vi "[ex ce] Signal Generation.vi"() -> ()   [LabVIEW 2021]
doc: "This simple example VI demonstrates a use of CalcExpress for signal generation. Resulting signal is played on a sound output device.\n\nYou need the <B>LabVIEW Advanced Analysis VIs</B> to run some scripts in this example VI.\n\n::: CalcExpress Toolkit :::\nCopyright (c) 2000-2026 Konstantin Shifershteyn. All rights reserved."
uses:
  <vilib>/sound2/lvsound2.llb/Sound Data Format.ctl
  <vilib>/sound2/lvsound2.llb/Sound Output Write (DBL Single).vi
panel:
  out "graph":dbl[](graph)
  in  "result variable":string="out"
  in  "Sound Rate (Hz) : rate":enum16{"11025", "22050", "44100"}(ring)
  in  "Sound device":u32
  in  "script selector":u16(ring) items=["***  Click here to select an example script  ***", "Sine Wave", "Beeper", "Damped oscillations"]
  in  "script":string="/*\nStart this VI and select an example script in the ring above for placing it into this text box.\n\nClick Exec button to process a script.\n*/\n"
  in  "stop":bool
  # "NOTE. Some functions of this example use Advanced Analysis VIs.\nThe example doesn't work properly if you don't have these VIs."
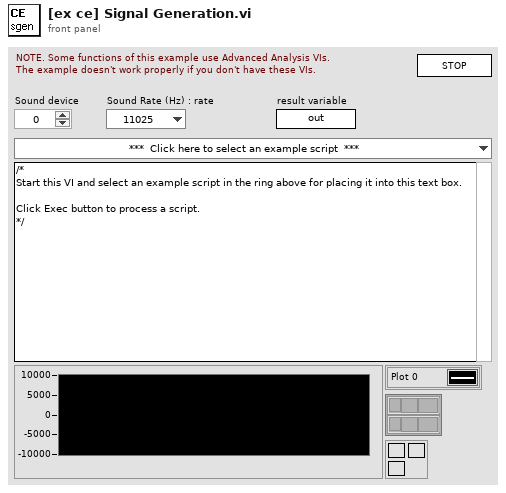
[diagram p1: front panel]
types:
  T1 = typedef "Sound Data Format.ctl" = cluster{"sample rate (S/s)":dbl, "number of channels":i32, "bits per sample":i32}
  T2 = enum16{"create", "destroy", "set value", "get value"}
  T3 = typedef "VarMan Variable Context Handle.ctl" = i32
  T4 = typedef "Sound Output Task ID.ctl" = u32
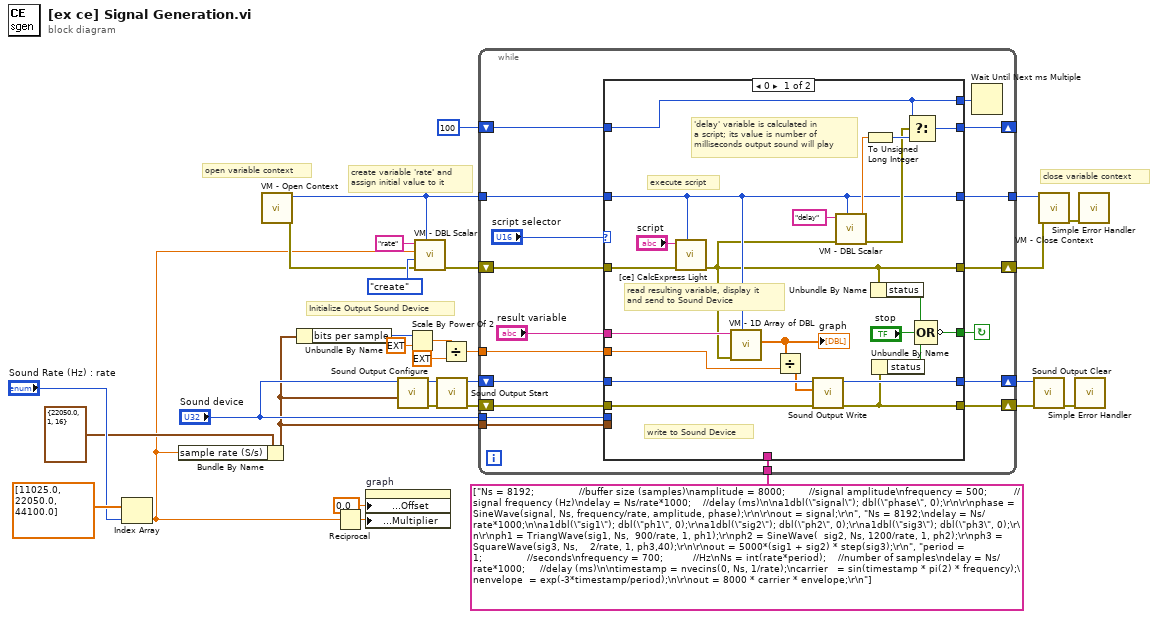
[diagram p0: block diagram]
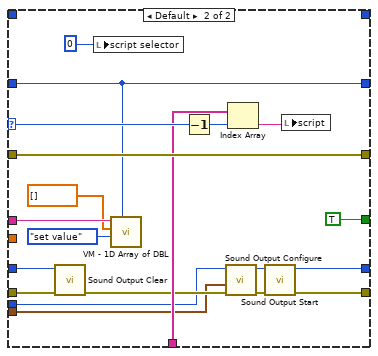
[diagram p2: hidden frame]
diagram:
  # "Initialize Output Sound Device"
  # "close variable context"
  # "create variable 'rate' and\nassign initial value to it"
  # "open variable context"
  n1 = Index Array(array=dbl[] [11025.0, 22050.0, 44100.0], index="Sound Rate (Hz) : rate") -> (element=w8:dbl)
  n2 = Bundle By Name(cluster=T1 {"sample rate (S/s)"=22050.0, "number of channels"=1, "bits per sample"=16} ("sound format"), "sample rate (S/s)"=w8) -> (w1:T1)
  n3 = call "VM - Open Context.vi"() -> ("error out"=w10:errorcluster, "VC Handle out"=w11:T3)  [unwired: 9 in, 1 out]
  n4 = Unbundle By Name(w1) -> ("bits per sample"=w7:i32)
  n5 = Reciprocal(x=w8) -> (1/x=w16:dbl)
  n6 = property on="graph" class="WFGraph (strict)"("X Scale.Offset and Multiplier:Offset"=0.0 ("Xo"), "X Scale.Offset and Multiplier:Multiplier"=w16) -> ()  [unwired: 2 in, 2 out]
  n7 = call <vilib>:"Sound Output Configure.vi"("sound format"=w1, "device ID"="Sound device") -> ("error out"=w19:errorcluster, "task ID"=w22:T4)  [unwired: 8 in]
  n8 = Scale By Power Of 2(n=w7, x=ext 1.0) -> (x*2^n=w5:ext)
  n9 = call "VM - DBL Scalar.vi"("VC Handle"=w11, "error in"=w10, "cmd"=T2."create", "value in"=w8, "name_spec"="rate" ("name")) -> ("error out"=w29:errorcluster)  [unwired: 1 in, 5 out]
  n10 = call <vilib>:"Sound Output Start.vi"("error in (no error)"=w19, "task ID"=w22) -> ("error out"=w20:errorcluster, "task ID out"=w21:T4)  [unwired: 8 in]
  n11 = Divide(x=w5, y=ext 2.0) -> (x/y=w4:ext)
  n12 = while {
    tunnel: string[] ["Ns = 8192;               //buffer size (samples)\namplitude = 8000;        //signal amplitude\nfrequency = 500;         //signal frequency (Hz)\ndelay = Ns/rate*1000;    //delay (ms)\n\na1dbl(\"signal\"); dbl(\"phase\", 0);\r\n\r\nphase = SineWave(signal, Ns, frequency/rate, amplitude, phase);\r\n\r\nout = signal;\r\n", "Ns = 8192;\ndelay = Ns/rate*1000;\n\na1dbl(\"sig1\"); dbl(\"ph1\", 0);\r\na1dbl(\"sig2\"); dbl(\"ph2\", 0);\r\na1dbl(\"sig3\"); dbl(\"ph3\", 0);\r\n\r\nph1 = TriangWave(sig1, Ns,  900/rate, 1, ph1);\r\nph2 = SineWave(  sig2, Ns, 1200/rate, 1, ph2);\r\nph3 = SquareWave(sig3, Ns,    2/rate, 1, ph3,40);\r\n\r\nout = 5000*(sig1 + sig2) * step(sig3);\r\n", "period = 1;               //seconds\nfrequency = 700;          //Hz\nNs = int(rate*period);    //number of samples\ndelay = Ns/rate*1000;     //delay (ms)\n\ntimestamp = nvecins(0, Ns, 1/rate);\ncarrier   = sin(timestamp * pi(2) * frequency);\nenvelope  = exp(-3*timestamp/period);\n\r\nout = 8000 * carrier * envelope;\r\n"] -> [w38]
    shift-left: u32 100 -> [w40]
    shift-right: [w41] -> _
    shift-left: w20 -> [w35]
    shift-right: [w43] -> w23
    tunnel: w11 -> [w47]
    tunnel: [w44] -> w30
    shift-left: w29 -> [w46]
    shift-right: [w42] -> w14
    tunnel: w4 -> [w37]
    shift-right: [w45] -> w24
    shift-left: w21 -> [w36]
    tunnel: "Sound device" -> [w33]
    tunnel: w1 -> [w32]
    stop <- w48 continue-if-true
    n13 = case shown="0" "script selector" {
      selector: "script selector" -> [_ w87]
      tunnel: [w70 TRUE] -> w48
      tunnel: w47 -> [w50 w74]
      tunnel: w46 -> [w68 w90]
      tunnel: w36 -> [w67 w82]
      tunnel: w35 -> [w66 w81]
      tunnel: [w65 w78] -> w45
      tunnel: [w50 w74] -> w44
      tunnel: [w63 w79] -> w43
      tunnel: [w49 w90] -> w42
      tunnel: [w58 _] -> w41
      tunnel: w40 -> [w57 _]
      tunnel: [w57 _] -> w39
      tunnel: w38 -> [_ w85]
      tunnel: w37 -> [w53 _]
      tunnel: w33 -> [_ w77]
      tunnel: w32 -> [_ w76]
      tunnel: "result variable" -> [w51 w75]
      frame 0 {
        # "'delay' variable is calculated in\na script; its value is number of\nmilliseconds output sound will play"
        # "read resulting variable, display it\nand send to Sound Device"
        # "execute script"
        # "write to Sound Device"
        n14 = call "[ce] CalcExpress Light.vi"("VC Handle"=w50, "error in"=w68, "expression"="script") -> ("error out"=w49:errorcluster)  [unwired: 6 in, 2 out]
        n15 = call "VM - 1D Array of DBL.vi"("VC Handle"=w50, "error in"=w49, "name_spec"=w51) -> ("value out"=w54:dbl[])  [unwired: 3 in, 5 out]
        "graph" <- w54
        n16 = Divide(x=w54, y=w53) -> (x/y=w52:ext[])
        n17 = call-poly <vilib>:"Sound Output Write.vi"("error in (no error)"=w66, "data"=w52, "task ID"=w67) -> ("error out"=w63:errorcluster, "task ID out"=w65:T4)  [unwired: 7 in]
        n18 = call "VM - DBL Scalar.vi"("VC Handle"=w50, "error in"=w49, "name_spec"="delay" ("name in")) -> ("error out"=w55:errorcluster, "value out"=w60:dbl)  [unwired: 3 in, 4 out]
        n19 = To Unsigned Long Integer(number=w60) -> (unsigned 32bit integer=w59:u32)
        n20 = Unbundle By Name(w49) -> ("status"=w56:bool)
        n21 = Unbundle By Name(w63) -> ("status"=w62:bool)
        n22 = Select(t=w57, s=w55, f=w59) -> (s? t:f=w58:u32)
        n23 = Compound Arithmetic op=OR(w56, "stop", w62) -> (invert w70:bool)
      }
      frame Default {
        n24 = call <vilib>:"Sound Output Clear.vi"("error in (no error)"=w81, "task ID"=w82) -> ("error out"=w80:errorcluster)  [unwired: 9 in]
        n25 = local write "script selector"(u16 0) -> ()
        n26 = call "VM - 1D Array of DBL.vi"("VC Handle"=w74, "cmd"=T2."set value", "value in"=dbl[] [], "name_spec"=w75) -> ()  [unwired: 2 in, 6 out]
        n27 = Decrement(x=w87) -> (x-1=w86:u16)
        n28 = call <vilib>:"Sound Output Configure.vi"("error in (no error)"=w80, "sound format"=w76, "device ID"=w77) -> ("error out"=w84:errorcluster, "task ID"=w83:T4)  [unwired: 7 in]
        n29 = Index Array(array=w85, index=w86) -> (element=w88:string)
        n30 = call <vilib>:"Sound Output Start.vi"("error in (no error)"=w84, "task ID"=w83) -> ("error out"=w79:errorcluster, "task ID out"=w78:T4)  [unwired: 8 in]
        n31 = local write "script"(w88) -> ()
      }
    }
    n32 = Wait Until Next ms Multiple(millisecond multiple=w39) -> ()  [unwired: 1 out]
  }
  n33 = call <vilib>:"Sound Output Clear.vi"("error in (no error)"=w23, "task ID"=w24) -> ("error out"=w18:errorcluster)  [unwired: 9 in]
  n34 = call "VM - Close Context.vi"("error in"=w14, "VC Handle"=w30) -> ("error out"=w13:errorcluster)  [unwired: 8 in, 1 out]
  n35 = call <vilib>:"Simple Error Handler.vi"("error in (no error)"=w18) -> ()  [unwired: 4 in, 5 out]
  n36 = call <vilib>:"Simple Error Handler.vi"("error in (no error)"=w13) -> ()  [unwired: 4 in, 5 out]
